vi "Write GUID.vi"(8 "error in (no error)":errorcluster, 10 "GUID":string, 11 "OOBgRPCService in":refnum<class "OOBgRPCService.lvclass">) -> (0 "error out":errorcluster, 3 "OOBgRPCService out":refnum<class "OOBgRPCService.lvclass">)   [LabVIEW 2025, in "OOB gRPC Server.lvlib" / "OOBgRPCService.lvclass"]
uses:
  OOBgRPCService.lvclass
  OOBgRPCService.lvclass/OOBgRPCService.ctl
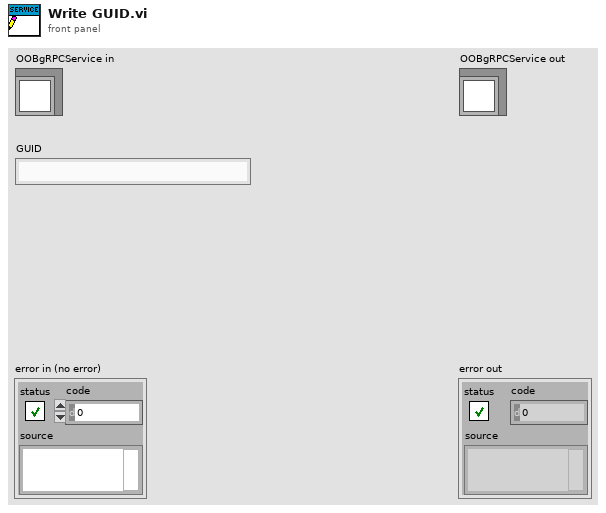
[diagram p1: front panel]
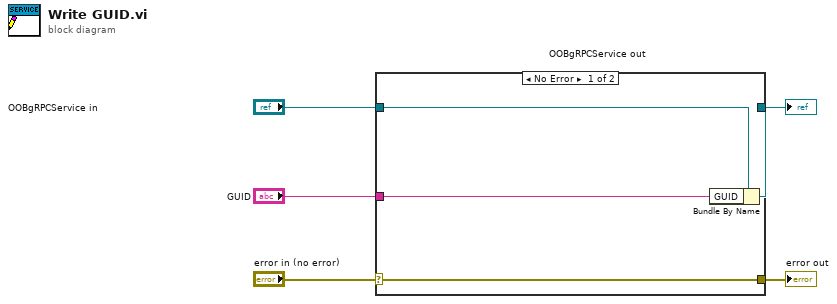
[diagram p0: block diagram]
diagram:
  n1 = case shown="No Error" "error in (no error)" {
    selector: "error in (no error)" -> [w9 w10]
    tunnel: [w9 w10] -> w4
    tunnel: [w7 w11] -> w2
    tunnel: "OOBgRPCService in" -> [w8 w11]
    tunnel: "GUID" -> [w6 _]
    frame No Error {
      n2 = Bundle By Name(cluster=w8, "GUID"=w6) -> (w7:refnum<class "OOBgRPCService.lvclass">)
    }
    frame Error {
    }
  }
  "error out" <- w4
  "OOBgRPCService out" <- w2
